vi "Migrate all Measurement Dependencies.vi"(0 "Project path":path, 1 "Measurement paths":path[](array[path]), 5 "Plug-in names":string[](array[string]), 7 "Measurement dependencies":path[][](array[path]), 9 "Outside items":string[](array[string]), 11 "error in (no error)":errorcluster, 12 "Shared dependent VIs":path[](array[path])) -> (6 "DestinationDirectory":path[](array[path]), 15 "error out":errorcluster)   [LabVIEW 2021, in "Multiple Migrator.lvlib"]
uses:
  Multiple Migrator.lvlib
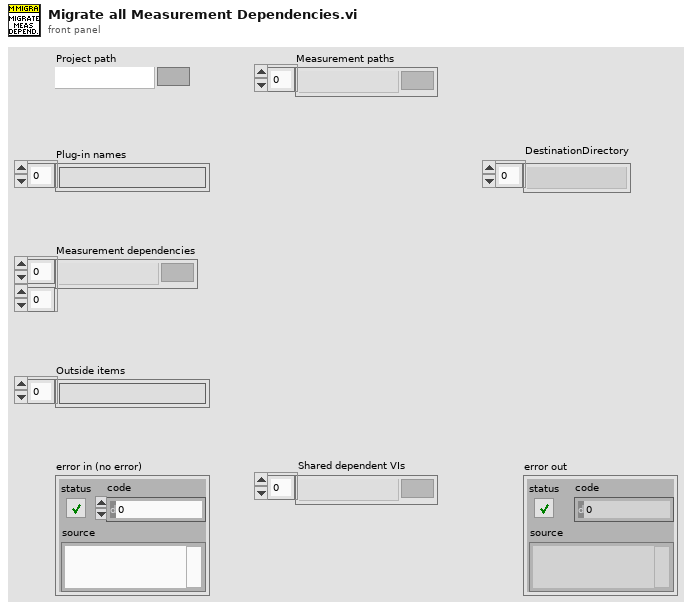
[diagram p1: front panel]
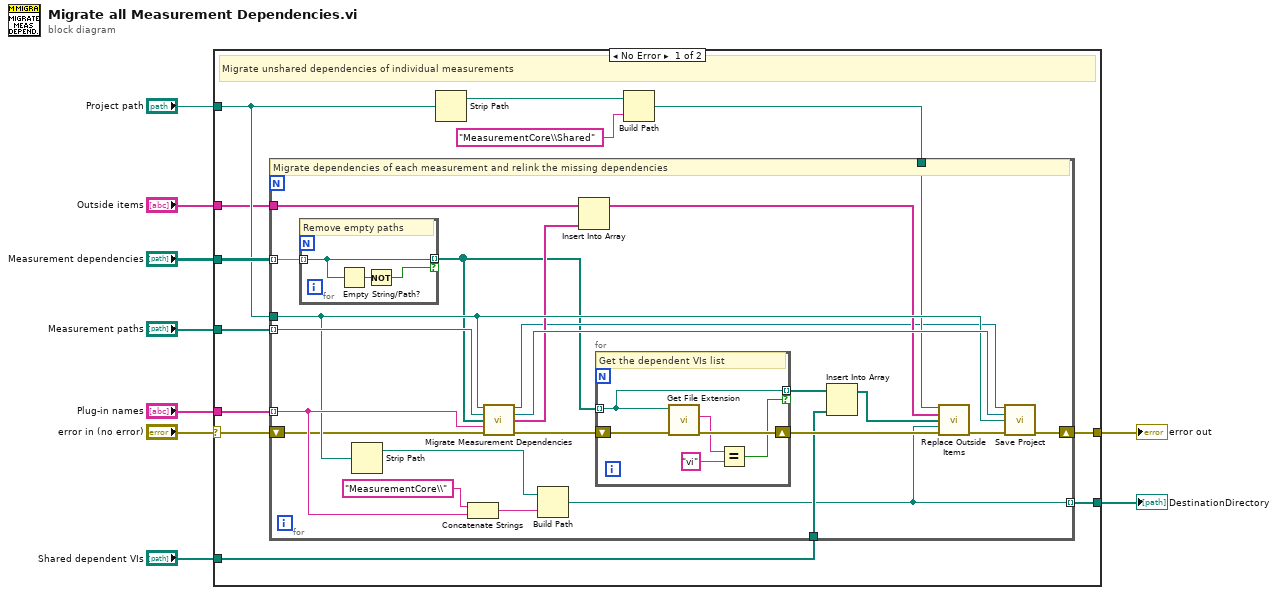
[diagram p0: block diagram]
diagram:
  n1 = case shown="No Error" "error in (no error)" {
    selector: "error in (no error)" -> [w20 w54]
    tunnel: "Measurement dependencies" -> [w21 _]
    tunnel: "Project path" -> [w16 _]
    tunnel: "Outside items" -> [w15 _]
    tunnel: "Measurement paths" -> [w14 _]
    tunnel: "Plug-in names" -> [w13 _]
    tunnel: [w12 w54] -> w3
    tunnel: "Shared dependent VIs" -> [w11 _]
    tunnel: [w10 _] -> w1
    frame No Error {
      # "Migrate unshared dependencies of individual measurements"
      n2 = Strip Path(path=w16) -> (stripped path=w17:path)  [unwired: 1 out]
      n3 = Build Path(base path=w17, name or relative path="MeasurementCore\\Shared" ("string")) -> (appended path=w19:path)
      n4 = for {
        tunnel: w16 -> [w36]
        tunnel: w14 -> [w41] mode=indexing
        tunnel: w13 -> [w38] mode=indexing
        tunnel: w15 -> [w35]
        tunnel: w19 -> [w32]
        shift-right: [w42] -> w12
        shift-left: w20 -> [w30]
        tunnel: w21 -> [w29] mode=indexing
        tunnel: w11 -> [w24]
        tunnel: [w22] -> w10 mode=indexing
        # "Migrate dependencies of each measurement and relink the missing dependencies"
        n5 = for {
          tunnel: w29 -> [w52] mode=indexing
          tunnel: [w52] -> w26 mode=indexing if=w51
          # "Remove empty paths"
          n6 = Empty String/Path?(string/path=w52) -> (empty?=w53:bool)
          n7 = Not(x=w53) -> (.not. x?=w51:bool)
        }
        n8 = Strip Path(path=w36) -> (stripped path=w37:path)  [unwired: 1 out]
        n9 = Concatenate Strings("MeasurementCore\\" ("string"), w38) -> (w27:string)
        n10 = call "Migrate Measurement Dependencies.vi"("Project path"=w36, "Measurement path"=w41, "Dependencies path"=w26, "Plug-in name"=w38, "error in (no error)"=w30) -> ("Project reference"=w31:refnum<vi>, "MeasurementCore reference"=w40:refnum<vi>, "Outside items"=w34:string[], "error out"=w44:errorcluster)  [unwired: 7 in]
        n11 = Build Path(base path=w37, name or relative path=w27) -> (appended path=w22:path)
        n12 = Insert Into Array(array=w35, new element=w34) -> (w33:string[])  [unwired: 1 in]
        n13 = for {
          shift-right: [w49] -> w28
          shift-left: w44 -> [w50]
          tunnel: w26 -> [w48] mode=indexing
          tunnel: [w48] -> w25 mode=indexing if=w45
          # "Get the dependent VIs list"
          n14 = call <vilib>:"Get File Extension.vi"("error in (no error)"=w50, "file"=w48) -> ("error out"=w49:errorcluster, "lowercase file extension"=w46:string)  [unwired: 5 in, 3 out]
          n15 = Equal?(x=w46, y="vi" ("x")) -> (x = y?=w45:bool)
        }
        n16 = Insert Into Array(array=w25, new element=w24) -> (w23:path[])  [unwired: 1 in]
        n17 = call "Replace Outside Items.vi"("Shared directory"=w32, "OutsideVIs"=w33, "Dependent VIs"=w23, "Measurement directory"=w22, "error in (no error)"=w28) -> ("error out"=w43:errorcluster)  [unwired: 10 in]
        n18 = call "Save Project.vi"("Project reference"=w31, "MeasurementCore reference"=w40, "Project path"=w36, "error in (no error)"=w43) -> ("error out"=w42:errorcluster)  [unwired: 11 in]
      }
    }
    frame Error {
      # "Pass"
    }
  }
  "error out" <- w3
  "DestinationDirectory" <- w1
